vi "Update Test-Assertion Measurement.vi"(8 "error in (no error)":errorcluster, 9 "Measurement":refnum<class "TestManagerMsg.Measurement.lvclass">, 11 "Test Event Storage in":refnum<class "Test Event Storage.lvclass">) -> (0 "error out":errorcluster, 3 "Test Event Storage out":refnum<class "Test Event Storage.lvclass">)   [LabVIEW 2020, in "Caraya.lvlib" / "Test Event Storage.lvclass"]
uses:
  Test Event Storage.lvclass
  Test Manager Message Measurement/TestManagerMsg.Measurement.lvclass
  C:/projects/caraya/src/classes/Test Manager Message/TestManagerMsg.lvclass
  Test Event Storage.lvclass/Test Event Storage.ctl
  assert store -- cluster.ctl
  Test Manager Message Assertion/TestManagerMsg.Assertion.lvclass
  Test Manager Message Verbose/TestManagerMsg.Verbose.lvclass
  Test Manager Message/TestManagerMsg.lvclass/TestManagerMsg.ctl
  Test Manager Message Measurement/TestManagerMsg.Measurement.lvclass/TestManagerMsg.Measurement.ctl
  Test Manager Message/TestManagerMsg.lvclass
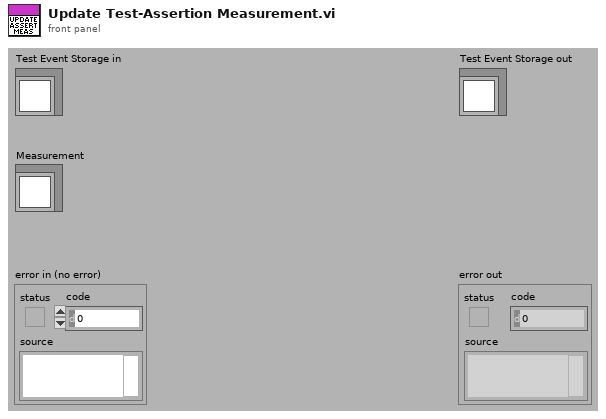
[diagram p1: front panel]
types:
  T1 = typedef "Caraya.lvlib/Test Event Storage.lvclass/assert store -- cluster.ctl" = cluster{"Assertion":refnum<class "TestManagerMsg.Assertion.lvclass">, "Explanation":refnum<class "TestManagerMsg.Verbose.lvclass">, "properties":variant, "measurements":variant, "user-defined":variant}
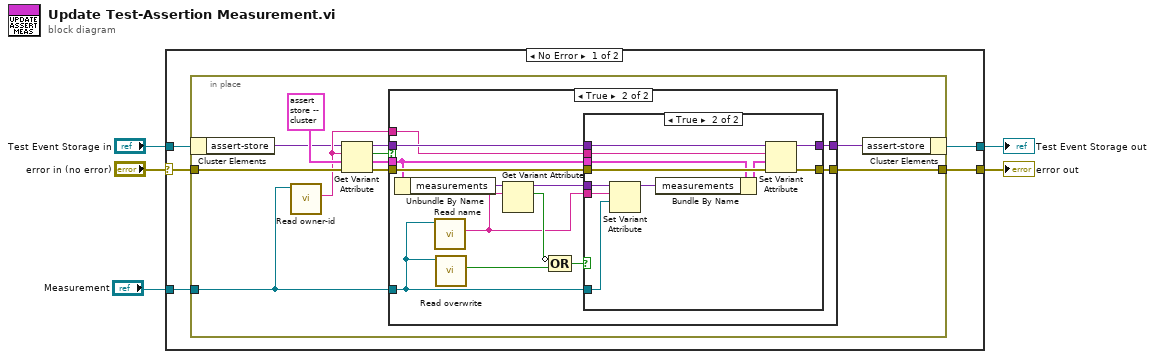
[diagram p0: block diagram]
diagram:
  n1 = case shown="No Error" "error in (no error)" {
    selector: "error in (no error)" -> [w8 w51]
    tunnel: [w10 w51] -> w4
    tunnel: [w9 w50] -> w2
    tunnel: "Test Event Storage in" -> [w6 w50]
    tunnel: "Measurement" -> [w7 _]
    frame No Error {
      n2 = in-place {
        in-place-border: w8 -> [w19]
        in-place-border: [w20] -> w10
        in-place-border: w7 -> [w18]
        n3 = in-place-cluster #1(w6) -> ("assert-store"=w11:variant)
        n4 = call "Read owner-id.vi"("TestManagerMsg in"=w18) -> ("owner-id"=w12:string)  [unwired: 9 in, 1 out]
        n5 = Get Variant Attribute(Variant=w11, name=w12, default value (empty Variant)=T1 {"Assertion"=refnum, "Explanation"=refnum, "properties"=variant, "measurements"=variant, "user-defined"=variant} ("assert-store"), error in=w19) -> (duplicate Variant=w17:variant, found=w16:bool, value=w15:T1, error out=w14:errorcluster)
        n6 = case shown="True" w16 {
          tunnel: [w23 w36] -> w21
          tunnel: [w22 w35] -> w20
          tunnel: w14 -> [w22 w34]
          tunnel: w17 -> [w23 w33]
          tunnel: w12 -> [_ w32]
          tunnel: w15 -> [_ w31]
          tunnel: w18 -> [_ w25]
          frame False {
          }
          frame True {
            n7 = Unbundle By Name(w31) -> ("measurements"=w29:variant)
            n8 = call "Read name.vi"("TestManagerMsg.Measurement in"=w25) -> ("name"=w24:string)  [unwired: 9 in, 1 out]
            n9 = call "Read overwrite.vi"("TestManagerMsg in"=w25) -> ("overwrite?"=w27:bool)  [unwired: 9 in, 1 out]
            n10 = Get Variant Attribute(Variant=w29, name=w24) -> (duplicate Variant=w26:variant, found=w28:bool)  [unwired: 2 in, 2 out]
            n11 = Compound Arithmetic op=OR(invert w28, w27) -> (w30:bool)
            n12 = case shown="True" w30 {
              tunnel: [w38 w49] -> w36
              tunnel: [w37 w48] -> w35
              tunnel: w34 -> [w37 w47]
              tunnel: w33 -> [w38 w46]
              tunnel: w32 -> [_ w45]
              tunnel: w31 -> [_ w44]
              tunnel: w25 -> [_ w39]
              tunnel: w26 -> [_ w41]
              tunnel: w24 -> [_ w40]
              frame False {
              }
              frame True {
                n13 = Set Variant Attribute(Variant=w41, name=w40, value=w39) -> (Variant out=w42:variant)  [unwired: 1 in, 2 out]
                n14 = Bundle By Name(cluster=w44, "measurements"=w42) -> (w43:T1)
                n15 = Set Variant Attribute(Variant=w46, name=w45, value=w43, error in=w47) -> (Variant out=w49:variant, error out=w48:errorcluster)  [unwired: 1 out]
              }
            }
          }
        }
        n16 = in-place-cluster #1("assert-store"=w21) -> (w9:refnum<class "Test Event Storage.lvclass">)
      }
    }
    frame Error {
    }
  }
  "error out" <- w4
  "Test Event Storage out" <- w2
